vi "1or2.vi"(11 "活动单元格:位置":T1 caption="位置") -> (3 "1/2":bool)   [LabVIEW 2025]
uses:
  <vilib>/Utility/miscctls.llb/LVPositionTypeDef.ctl
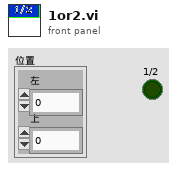
[diagram p1: front panel]
types:
  T1 = typedef "LVPositionTypeDef.ctl" = cluster{"Left":i32, "Top":i32}
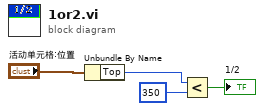
[diagram p0: block diagram]
diagram:
  n1 = Unbundle By Name("活动单元格:位置") -> ("Top"=w3:i32)
  n2 = Less?(x=w3, y=350) -> (x < y?=→"1/2":bool)
